vi "Report Digital Command.vi"(6 "Value":bool, 8 "error in (no error)":errorcluster, 9 "Name":string, 10 "VolatusAPI in":refnum<class "VolatusAPI.lvclass">, 11 "GUI Element in":refnum<class "GUI Element.lvclass">) -> (0 "error out":errorcluster, 3 "GUI Element out":refnum<class "GUI Element.lvclass">)   [LabVIEW 2020, in "VolatusGUI.lvlib" / "GUI Element.lvclass"]
uses:
  GUI Element.lvclass
  Volatus/VolatusAPI/VolatusAPI.lvclass
  GUI Element.lvclass/GUI Element.ctl
  lv-vecto/Vecto/Vecto.lvlib
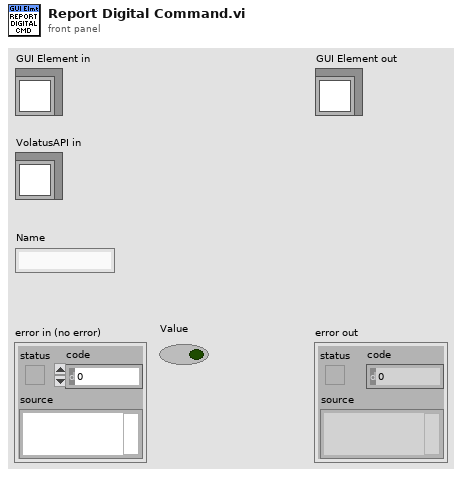
[diagram p1: front panel]
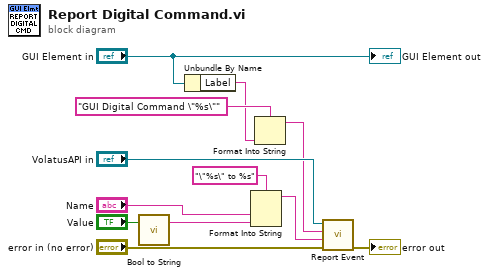
[diagram p0: block diagram]
diagram:
  n1 = call "Bool to String.vi"("Bool"="Value") -> ("String"=w8:string)  [unwired: 2 in]
  n2 = Unbundle By Name("GUI Element in") -> ("Label"=w2:string)
  n3 = Format Into String(format string="\"%s\" to %s", "Name", w8) -> (resulting string=w6:string)  [unwired: 2 in, 1 out]
  n4 = Format Into String(format string="GUI Digital Command \"%s\"" ("string"), w2) -> (resulting string=w1:string)  [unwired: 2 in, 1 out]
  n5 = call "Report Event.vi"("error in (no error)"="error in (no error)", "Message"=w6, "Context"=w1, "VolatusAPI in"="VolatusAPI in") -> ("error out"=→"error out":errorcluster)  [unwired: 6 in, 1 out]
  "GUI Element out" <- "GUI Element in"
